vi "OverlayFeaturePoints.vi"(4 "Color":u32(colorbox)=16711680, 6 "FeaturePointStyle":T1, 7 "GroupName":string, 8 "error in":errorcluster, 9 "Size":i32=10, 10 "FeaturePoint":T2[](array[typedef]), 11 "Image Reference In":T3) -> (0 "error out":errorcluster, 3 "Image Reference Out":T3)   [LabVIEW 2020, in "OpenLvVision_Overlays.lvlib"]
doc: "Overlay of feature points.\nYou can select the style and size."
uses:
  OpenLvVision_Overlays.lvlib
  <vilib>/OpenLvVision/OpenLvVision_Image/Management/TypeDef/OLV Image.ctl
  TypeDefs/PointI32.ctl
  TypeDefs/FeaturePointStyle.ctl
  TypeDefs/DrawingMode.ctl
  <vilib>/OpenLvVision/OpenLvVision_Image/Management/OLV Management.lvlib
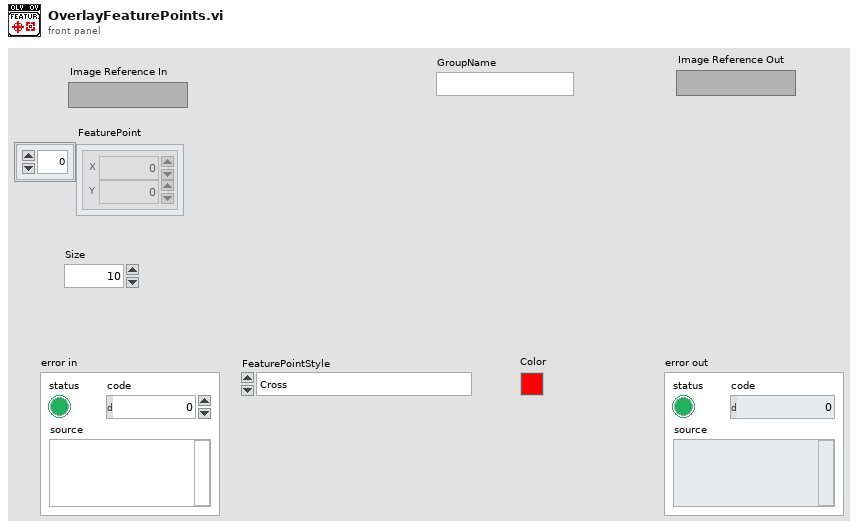
[diagram p1: front panel]
types:
  T1 = typedef "OpenLvVision_Overlays.lvlib/FeaturePointStyle.ctl" = enum16{"Cross", "TiltedCross", "Star", "Diamond", "Square", "TriangleUp", "TriangleDown", "Crosshair"}
  T2 = typedef "OpenLvVision_Overlays.lvlib/PointI32.ctl" = cluster{"X":i32, "Y":i32}
  T3 = typedef "OLV OpenLvVision_Image.lvlib/OLV Management.lvlib/OLV Image.ctl" = refnum<image>
  T4 = typedef "OpenLvVision_Overlays.lvlib/DrawingMode.ctl" = enum16{"Frame", "Fill"}
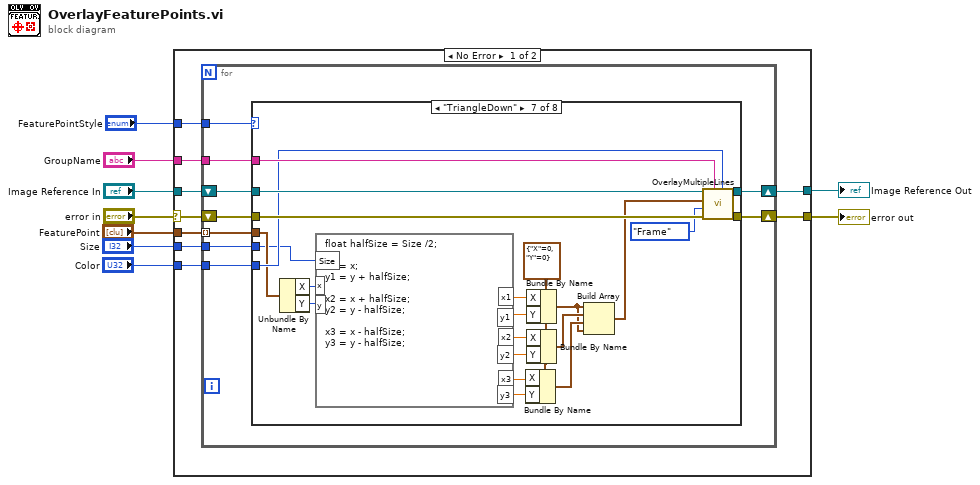
[diagram p0: block diagram]
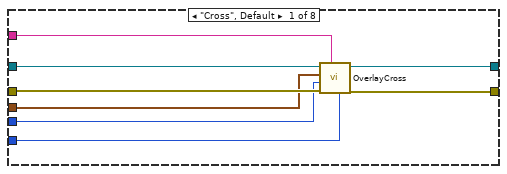
[diagram p2: hidden frame]
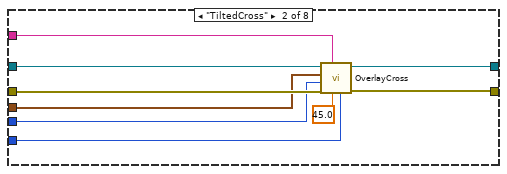
[diagram p3: hidden frame]
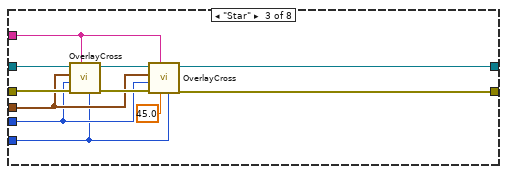
[diagram p4: hidden frame]
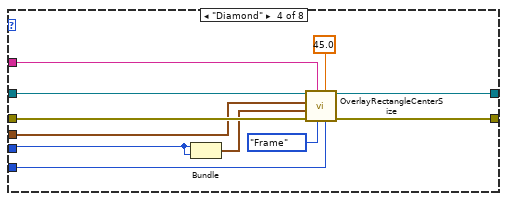
[diagram p5: hidden frame]
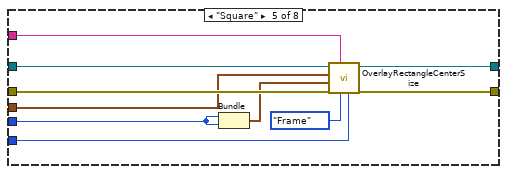
[diagram p6: hidden frame]
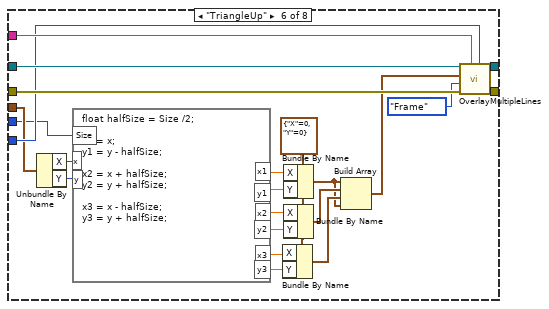
[diagram p7: hidden frame]
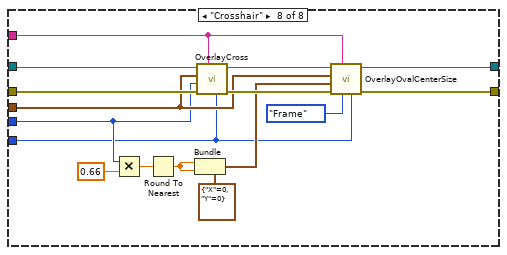
[diagram p8: hidden frame]
diagram:
  n1 = case shown="No Error" "error in" {
    selector: "error in" -> [w18 w137]
    tunnel: [w15 w137] -> w8
    tunnel: "Image Reference In" -> [w17 w138]
    tunnel: [w16 w138] -> w7
    tunnel: "GroupName" -> [w13 _]
    tunnel: "Color" -> [w12 _]
    tunnel: "Size" -> [w11 _]
    tunnel: "FeaturePointStyle" -> [w14 _]
    tunnel: "FeaturePoint" -> [w10 _]
    frame No Error {
      n2 = for {
        shift-right: [w20] -> w15
        shift-left: w18 -> [w24]
        shift-right: [w21] -> w16
        shift-left: w17 -> [w25]
        tunnel: w14 -> [w27]
        tunnel: w13 -> [w26]
        tunnel: w12 -> [w23]
        tunnel: w11 -> [w22]
        tunnel: w10 -> [w19] mode=indexing
        n3 = case shown="\"TriangleDown\"" w27 {
          tunnel: w26 -> [w31 w42 w45 w62 w74 w94 w116 w125]
          tunnel: w25 -> [w32 w41 w55 w63 w73 w95 w117 w126]
          tunnel: w24 -> [w33 w40 w54 w64 w72 w96 w118 w127]
          tunnel: w23 -> [w30 w38 w49 w59 w70 w92 w114 w121]
          tunnel: w22 -> [w29 w39 w50 w57 w68 w88 w110 w122]
          tunnel: [w35 w44 w47 w66 w76 w98 w120 w129] -> w21
          tunnel: [w34 w43 w46 w65 w75 w97 w119 w128] -> w20
          tunnel: w19 -> [w28 w37 w51 w61 w71 w91 w113 w123]
          frame "Cross", Default {
            n4 = call "OverlayCross.vi"("Color"=w30, "GroupName"=w31, "error in"=w33, "Size"=w29, "Point"=w28, "Image Reference In"=w32) -> ("error out"=w34:errorcluster, "Image Reference Out"=w35:T3)  [unwired: 4 in]
          }
          frame "TiltedCross" {
            n5 = call "OverlayCross.vi"("Color"=w38, "Angle"=45.0, "GroupName"=w42, "error in"=w40, "Size"=w39, "Point"=w37, "Image Reference In"=w41) -> ("error out"=w43:errorcluster, "Image Reference Out"=w44:T3)  [unwired: 3 in]
          }
          frame "Star" {
            n6 = call "OverlayCross.vi"("Color"=w49, "GroupName"=w45, "error in"=w54, "Size"=w50, "Point"=w51, "Image Reference In"=w55) -> ("error out"=w52:errorcluster, "Image Reference Out"=w53:T3)  [unwired: 4 in]
            n7 = call "OverlayCross.vi"("Color"=w49, "Angle"=45.0, "GroupName"=w45, "error in"=w52, "Size"=w50, "Point"=w51, "Image Reference In"=w53) -> ("error out"=w46:errorcluster, "Image Reference Out"=w47:T3)  [unwired: 3 in]
          }
          frame "Diamond" {
            n8 = Bundle("Size"=w57, "Size"=w57) -> (w56:cluster{"Size":i32, "Size":i32})  [unwired: 1 in]
            n9 = call "OverlayRectangleCenterSize.vi"("Color"=w59, "Angle"=45.0, "Drawing Mode (Frame)"=DrawingMode."Frame", "GroupName"=w62, "error in"=w64, "Size"=w56, "Center-Point"=w61, "Image Reference In"=w63) -> ("error out"=w65:errorcluster, "Image Reference Out"=w66:T3)  [unwired: 2 in]
          }
          frame "Square" {
            n10 = Bundle("Size"=w68, "Size"=w68) -> (w67:cluster{"Size":i32, "Size":i32})  [unwired: 1 in]
            n11 = call "OverlayRectangleCenterSize.vi"("Color"=w70, "Drawing Mode (Frame)"=DrawingMode."Frame", "GroupName"=w74, "error in"=w72, "Size"=w67, "Center-Point"=w71, "Image Reference In"=w73) -> ("error out"=w75:errorcluster, "Image Reference Out"=w76:T3)  [unwired: 3 in]
          }
          frame "TriangleUp" {
            w86 = T2 {"X"=0, "Y"=0} ("Point")
            n12 = Unbundle By Name(w91) -> ("X"=w90:i32, "Y"=w89:i32)
            n13 = formula code="float halfSize = Size /2;\n\nx1 = x;\ny1 = y - halfSize;\n\nx2 = x + halfSize;\ny2 = y + halfSize;\n\nx3 = x - halfSize;\ny3 = y + halfSize;"("x"=w90, "y"=w89, "Size"=w88) -> ("x1"=w83:dbl, "y1"=w84:dbl, "x2"=w82:dbl, "y2"=w81:dbl, "x3"=w80:dbl, "y3"=w79:dbl)
            n14 = Bundle By Name(cluster=w86, "X"=w80, "Y"=w79) -> (w78:T2)
            n15 = Bundle By Name(cluster=w86, "X"=w83, "Y"=w84) -> (w77:T2)
            n16 = Bundle By Name(cluster=w86, "X"=w82, "Y"=w81) -> (w87:T2)
            n17 = Build Array(w77, w87, w78, w77) -> (w85:T2[])
            n18 = call "OverlayMultipleLines.vi"("Color"=w92, "GroupName"=w94, "error in"=w96, "Drawing Mode (Frame)"=DrawingMode."Frame", "Points"=w85, "Image Reference In"=w95) -> ("error out"=w97:errorcluster, "Image Reference Out"=w98:T3)  [unwired: 4 in]
          }
          frame "TriangleDown" {
            w108 = T2 {"X"=0, "Y"=0} ("Point")
            n19 = Unbundle By Name(w113) -> ("X"=w112:i32, "Y"=w111:i32)
            n20 = formula code="float halfSize = Size /2;\n\nx1 = x;\ny1 = y + halfSize;\n\nx2 = x + halfSize;\ny2 = y - halfSize;\n\nx3 = x - halfSize;\ny3 = y - halfSize;"("x"=w112, "y"=w111, "Size"=w110) -> ("x1"=w105:dbl, "y1"=w106:dbl, "x2"=w104:dbl, "y2"=w103:dbl, "x3"=w102:dbl, "y3"=w101:dbl)
            n21 = Bundle By Name(cluster=w108, "X"=w102, "Y"=w101) -> (w100:T2)
            n22 = Bundle By Name(cluster=w108, "X"=w105, "Y"=w106) -> (w99:T2)
            n23 = Bundle By Name(cluster=w108, "X"=w104, "Y"=w103) -> (w109:T2)
            n24 = Build Array(w99, w109, w100, w99) -> (w107:T2[])
            n25 = call "OverlayMultipleLines.vi"("Color"=w114, "GroupName"=w116, "error in"=w118, "Drawing Mode (Frame)"=DrawingMode."Frame", "Points"=w107, "Image Reference In"=w117) -> ("error out"=w119:errorcluster, "Image Reference Out"=w120:T3)  [unwired: 4 in]
          }
          frame "Crosshair" {
            n26 = Multiply(x=w122, y=0.66) -> (x*y=w135:dbl)
            n27 = Round To Nearest(number=w135) -> (nearest integer value=w136:dbl)
            n28 = Bundle(cluster=T2 {"X"=0, "Y"=0} ("Size"), "X"=w136, "Y"=w136) -> (w124:T2)
            n29 = call "OverlayCross.vi"("Color"=w121, "GroupName"=w125, "error in"=w127, "Size"=w122, "Point"=w123, "Image Reference In"=w126) -> ("error out"=w134:errorcluster, "Image Reference Out"=w133:T3)  [unwired: 4 in]
            n30 = call "OverlayOvalCenterSize.vi"("Color"=w121, "Drawing Mode (Frame)"=DrawingMode."Frame", "GroupName"=w125, "error in"=w134, "Size"=w124, "Center-Point"=w123, "Image Reference In"=w133) -> ("error out"=w128:errorcluster, "Image Reference Out"=w129:T3)  [unwired: 3 in]
          }
        }
      }
    }
    frame Error {
    }
  }
  "error out" <- w8
  "Image Reference Out" <- w7
